vi "Close Connection.vi"(8 "error in (no error)":errorcluster, 11 "HID Handle":i64) -> (0 "error out":errorcluster)   [LabVIEW 2021, in "USB Relay Control.lvlib"]
uses:
  USB Relay Control.lvlib
  kernel32.dll
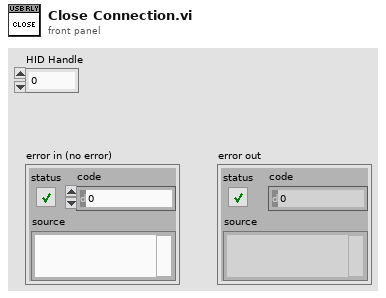
[diagram p1: front panel]
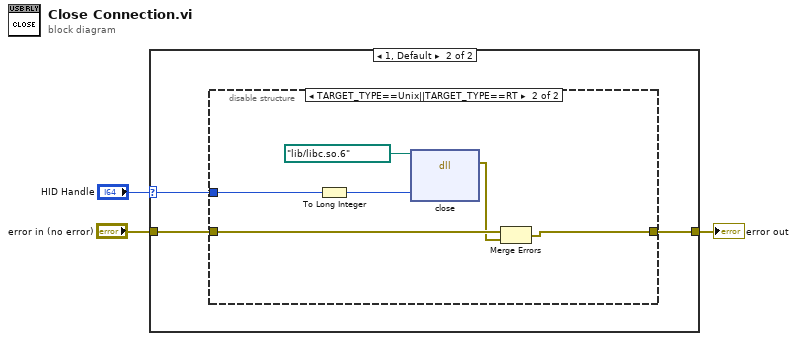
[diagram p0: block diagram]
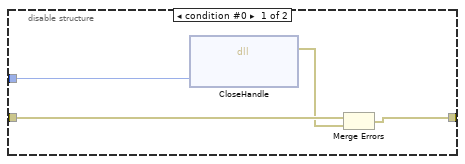
[diagram p3: hidden frame]
diagram:
  n1 = case shown="1, Default" "HID Handle" {
    selector: "HID Handle" -> [_ w5]
    tunnel: "error in (no error)" -> [w4 w7]
    tunnel: [w4 w6] -> w2
    frame 0 {
    }
    frame 1, Default {
      n2 = disable-structure shown="TARGET_TYPE==Unix||TARGET_TYPE==RT" {
        disable-tunnel: w7 -> [w11 w16]
        disable-tunnel: [w9 w14] -> w6
        disable-tunnel: w5 -> [w8 w13]
        frame condition #0 {
          n3 = dll-call lib="kernel32.dll" fn="CloseHandle"("hObject"=w8) -> (error out=w10:errorcluster)  [unwired: 5 in, 1 out]
          n4 = Merge Errors(w11, w10) -> (w9:errorcluster)
        }
        frame condition #1 (active) {
          n5 = To Long Integer(number=w13) -> (32bit integer=w12:i32)
          n6 = dll-call lib="lib/libc.so.6" fn="close"(path in=path "/lib/libc.so.6" ("librt path"), "fd"=w12) -> (error out=w15:errorcluster)  [unwired: 4 in, 1 out]
          n7 = Merge Errors(w16, w15) -> (w14:errorcluster)
        }
      }
    }
  }
  "error out" <- w2
